vi "midiInReset.vi"(8 "error in":errorcluster, 11 "midi in":refnum<class "midi.lvclass">) -> (0 "error out":errorcluster, 3 "midi out":refnum<class "midi.lvclass">)   [LabVIEW 2020, in "midi.lvclass"]
doc: "The midiInReset function stops input on a given MIDI input device.\n\nThis function returns all pending input buffers to the callback function and sets the MHDR_DONE flag in the dwFlags member of the MIDIHDR structure."
uses:
  midi.lvclass
  winmm.dll
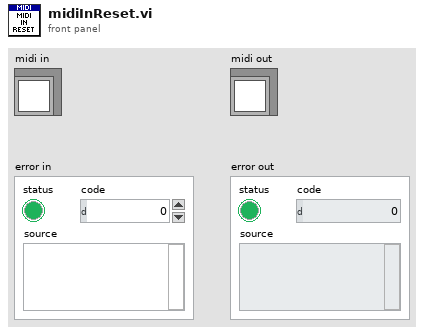
[diagram p1: front panel]
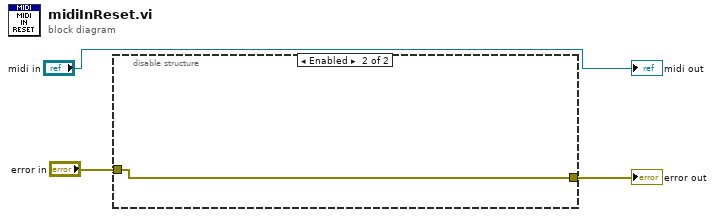
[diagram p0: block diagram]
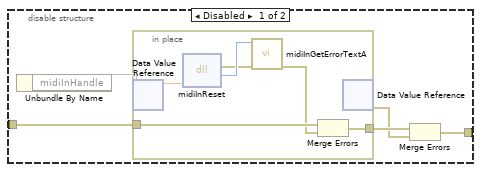
[diagram p2: hidden frame]
diagram:
  n1 = disable-structure shown="Enabled" {
    disable-tunnel: "error in" -> [w8 w16]
    disable-tunnel: [w4 w16] -> w2
    frame Disabled {
      n2 = Unbundle By Name() -> (w9:refnum<class "midi.lvclass">, "midiInHandle"=w7)
      n3 = in-place {
        in-place-border: w8 -> [w13]
        in-place-border: [w11] -> w6
        n4 = in-place-dvr #1(w7) -> (w10:dbl)  [unwired: 1 out]
        n5 = dll-call lib="winmm.dll" fn="midiInReset"("hmi"=w10) -> (error out=w14:errorcluster, "return type"=w15:i32)  [unwired: 4 in, 1 out]
        n6 = call "midiInGetErrorTextA.vi"("error in"=w14, "Error Code"=w15) -> ("error out"=w12:errorcluster)  [unwired: 9 in]
        n7 = Merge Errors(w13, w12) -> (w11:errorcluster)
        n8 = in-place-dvr #1() -> (w5:errorcluster)  [unwired: 1 in, 1 out]
      }
      n9 = Merge Errors(w6, w5) -> (w4:errorcluster)
    }
    frame Enabled {
    }
  }
  "error out" <- w2
  "midi out" <- "midi in"
